vi "Base species cluster.vi"(11 "Base":string) -> (0 "ex":string, 1 "Base Color":u32, 2 "Base Array":bool[](array[boolean]), 3 "Base Species IDX":i32, 4 "Item":T1)   [LabVIEW 2018]
panel:
  out "R STD Level":dbl
  out "R Base Level":dbl
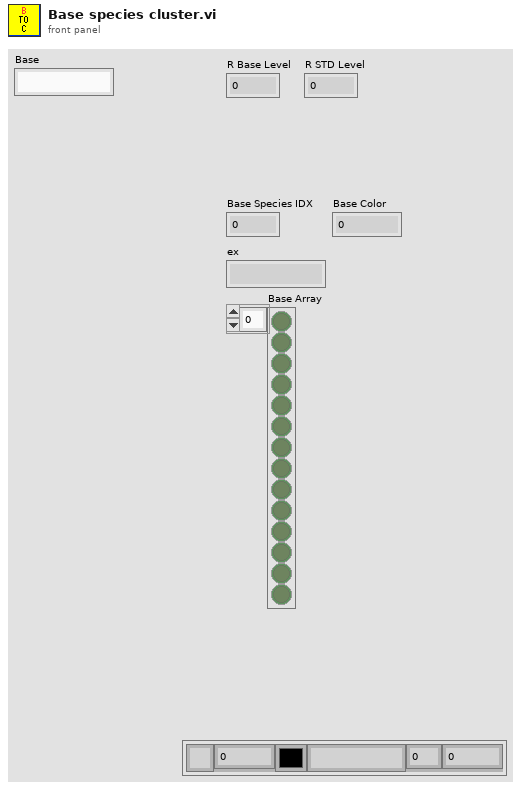
[diagram p1: front panel]
types:
  T1 = cluster{"Name":string, "Value":dbl, "Color":u32, "Name 2":string, "Value 2":dbl, "Value 3":dbl}
  T2 = cluster{"Base":string, dbl, u32, "y":string, i32, dbl}
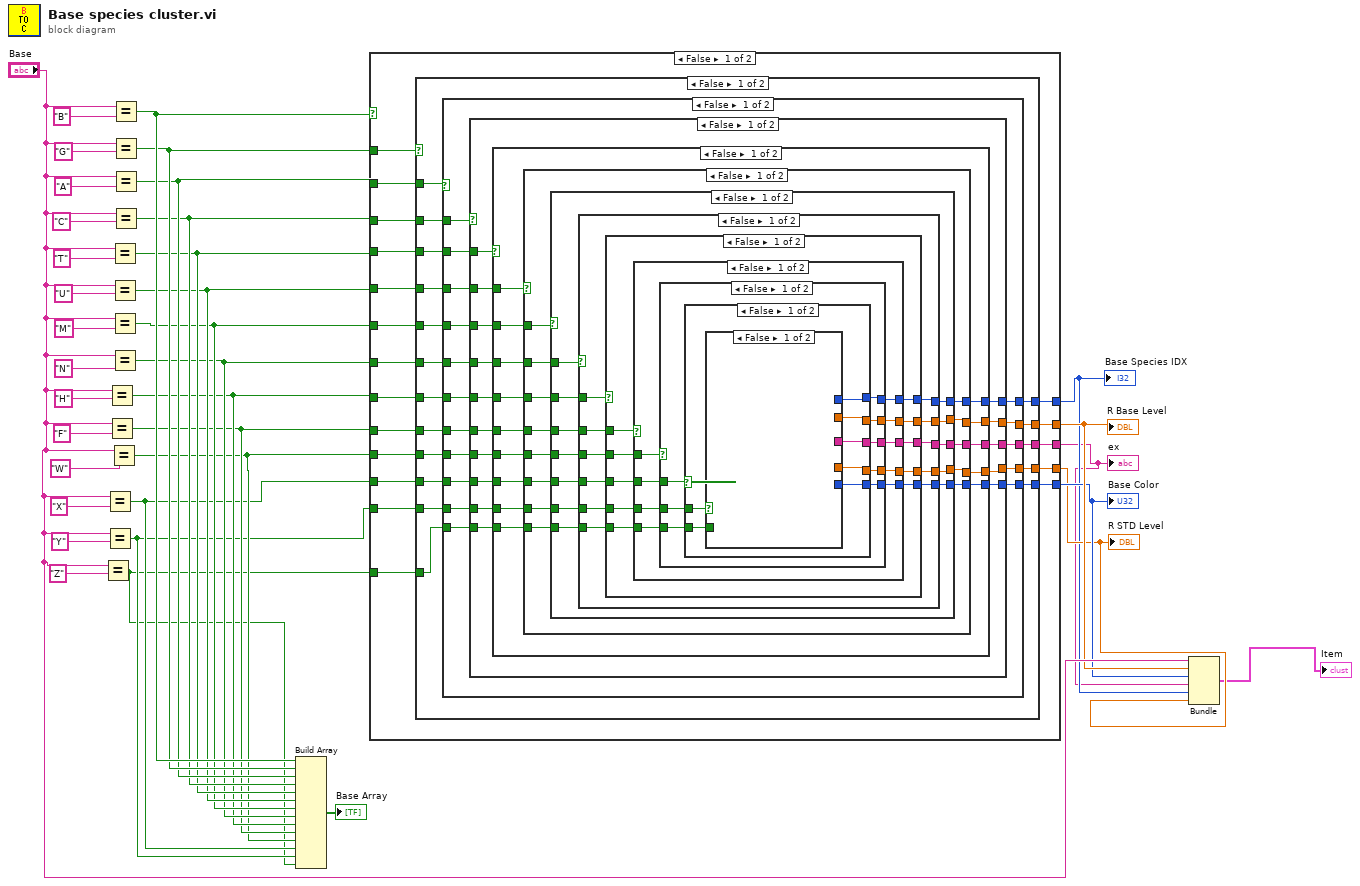
[diagram p0: block diagram]
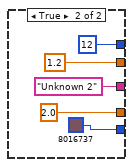
[diagram p2: hidden frame]
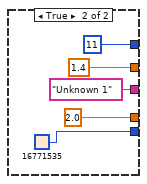
[diagram p3: hidden frame]
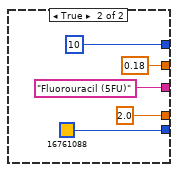
[diagram p4: hidden frame]
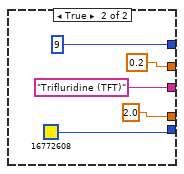
[diagram p5: hidden frame]
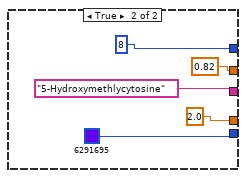
[diagram p6: hidden frame]
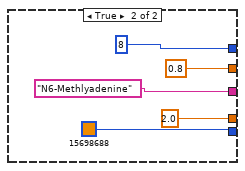
[diagram p7: hidden frame]
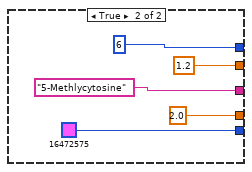
[diagram p8: hidden frame]
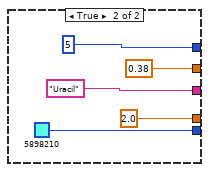
[diagram p9: hidden frame]
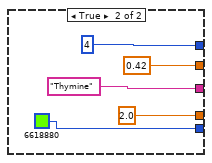
[diagram p10: hidden frame]
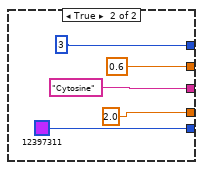
[diagram p11: hidden frame]
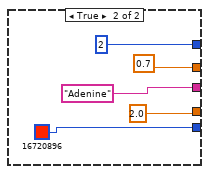
[diagram p12: hidden frame]
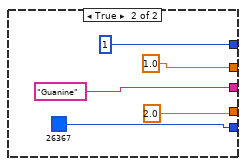
[diagram p13: hidden frame]
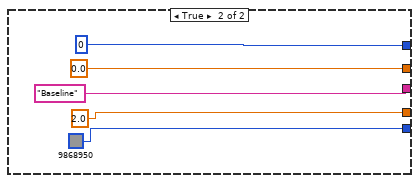
[diagram p14: hidden frame]
diagram:
  n1 = Equal?(x="Base", y="Z") -> (x = y?=w9:bool)
  n2 = Equal?(x="Base", y="X") -> (x = y?=w11:bool)
  n3 = Equal?(x="Base", y="Y") -> (x = y?=w10:bool)
  n4 = Equal?(x="Base", y="H") -> (x = y?=w14:bool)
  n5 = Equal?(x="Base", y="F") -> (x = y?=w13:bool)
  n6 = Equal?(x="Base", y="W") -> (x = y?=w12:bool)
  n7 = Equal?(x="Base", y="T") -> (x = y?=w18:bool)
  n8 = Equal?(x="Base", y="U") -> (x = y?=w17:bool)
  n9 = Equal?(x="Base", y="M") -> (x = y?=w16:bool)
  n10 = Equal?(x="Base", y="N") -> (x = y?=w15:bool)
  n11 = Equal?(x="Base", y="B") -> (x = y?=w22:bool)
  n12 = Equal?(x="Base", y="G") -> (x = y?=w21:bool)
  n13 = Equal?(x="Base", y="A") -> (x = y?=w20:bool)
  n14 = Equal?(x="Base", y="C") -> (x = y?=w19:bool)
  n15 = Build Array(w22, w21, w20, w19, w18, w17, w16, w15, w14, w13, w12, w11, w10, w9) -> (→"Base Array":bool[])
  n16 = case shown="False" w22 {
    tunnel: [w53 0] -> w3
    tunnel: w21 -> [w54 _]
    tunnel: [w52 "Baseline" ("y")] -> w2
    tunnel: w20 -> [w51 _]
    tunnel: w19 -> [w50 _]
    tunnel: w18 -> [w49 _]
    tunnel: w17 -> [w48 _]
    tunnel: w16 -> [w47 _]
    tunnel: w15 -> [w46 _]
    tunnel: w14 -> [w45 _]
    tunnel: w13 -> [w44 _]
    tunnel: w12 -> [w43 _]
    tunnel: w11 -> [w42 _]
    tunnel: w10 -> [w41 _]
    tunnel: w9 -> [w40 _]
    tunnel: [w39 u32 9868950] -> w5
    tunnel: [w38 0.0] -> w6
    tunnel: [w37 2.0] -> w4
    frame False {
      n17 = case shown="False" w54 {
        tunnel: [w71 1] -> w53
        tunnel: [w69 "Guanine" ("y")] -> w52
        tunnel: w51 -> [w70 _]
        tunnel: w50 -> [w68 _]
        tunnel: w49 -> [w67 _]
        tunnel: w48 -> [w66 _]
        tunnel: w47 -> [w65 _]
        tunnel: w46 -> [w64 _]
        tunnel: w45 -> [w63 _]
        tunnel: w44 -> [w62 _]
        tunnel: w43 -> [w61 _]
        tunnel: w42 -> [w60 _]
        tunnel: w41 -> [w59 _]
        tunnel: w40 -> [w58 _]
        tunnel: [w57 u32 26367] -> w39
        tunnel: [w56 1.0] -> w38
        tunnel: [w55 2.0] -> w37
        frame False {
          n18 = case shown="False" w70 {
            tunnel: [w86 2] -> w71
            tunnel: [w85 "Adenine" ("y")] -> w69
            tunnel: w68 -> [w87 _]
            tunnel: w67 -> [w84 _]
            tunnel: w66 -> [w83 _]
            tunnel: w65 -> [w82 _]
            tunnel: w64 -> [w81 _]
            tunnel: w63 -> [w80 _]
            tunnel: w62 -> [w79 _]
            tunnel: w61 -> [w78 _]
            tunnel: w60 -> [w77 _]
            tunnel: w59 -> [w76 _]
            tunnel: w58 -> [w75 _]
            tunnel: [w74 u32 16720896] -> w57
            tunnel: [w73 0.7] -> w56
            tunnel: [w72 2.0] -> w55
            frame False {
              n19 = case shown="False" w87 {
                tunnel: [w102 3] -> w86
                tunnel: [w100 "Cytosine"] -> w85
                tunnel: w84 -> [w101 _]
                tunnel: w83 -> [w99 _]
                tunnel: w82 -> [w98 _]
                tunnel: w81 -> [w97 _]
                tunnel: w80 -> [w96 _]
                tunnel: w79 -> [w95 _]
                tunnel: w78 -> [w94 _]
                tunnel: w77 -> [w93 _]
                tunnel: w76 -> [w92 _]
                tunnel: w75 -> [w91 _]
                tunnel: [w90 u32 12397311] -> w74
                tunnel: [w89 0.6] -> w73
                tunnel: [w88 2.0] -> w72
                frame False {
                  n20 = case shown="False" w101 {
                    tunnel: [w115 4] -> w102
                    tunnel: [w114 "Thymine"] -> w100
                    tunnel: w99 -> [w116 _]
                    tunnel: w98 -> [w113 _]
                    tunnel: w97 -> [w112 _]
                    tunnel: w96 -> [w111 _]
                    tunnel: w95 -> [w110 _]
                    tunnel: w94 -> [w109 _]
                    tunnel: w93 -> [w108 _]
                    tunnel: w92 -> [w107 _]
                    tunnel: w91 -> [w106 _]
                    tunnel: [w105 u32 6618880] -> w90
                    tunnel: [w104 0.42] -> w89
                    tunnel: [w103 2.0] -> w88
                    frame False {
                      n21 = case shown="False" w116 {
                        tunnel: [w128 5] -> w115
                        tunnel: [w127 "Uracil"] -> w114
                        tunnel: w113 -> [w129 _]
                        tunnel: w112 -> [w126 _]
                        tunnel: w111 -> [w125 _]
                        tunnel: w110 -> [w124 _]
                        tunnel: w109 -> [w123 _]
                        tunnel: w108 -> [w122 _]
                        tunnel: w107 -> [w121 _]
                        tunnel: w106 -> [w120 _]
                        tunnel: [w119 u32 5898210] -> w105
                        tunnel: [w118 0.38] -> w104
                        tunnel: [w117 2.0] -> w103
                        frame False {
                          n22 = case shown="False" w129 {
                            tunnel: [w140 6] -> w128
                            tunnel: [w139 "5-Methlycytosine"] -> w127
                            tunnel: w126 -> [w141 _]
                            tunnel: w125 -> [w138 _]
                            tunnel: w124 -> [w137 _]
                            tunnel: w123 -> [w136 _]
                            tunnel: w122 -> [w135 _]
                            tunnel: w121 -> [w134 _]
                            tunnel: w120 -> [w133 _]
                            tunnel: [w132 u32 16472575] -> w119
                            tunnel: [w131 1.2] -> w118
                            tunnel: [w130 2.0] -> w117
                            frame False {
                              n23 = case shown="False" w141 {
                                tunnel: [w151 8] -> w140
                                tunnel: [w150 "N6-Methlyadenine"] -> w139
                                tunnel: w138 -> [w152 _]
                                tunnel: w137 -> [w149 _]
                                tunnel: w136 -> [w148 _]
                                tunnel: w135 -> [w147 _]
                                tunnel: w134 -> [w146 _]
                                tunnel: w133 -> [w145 _]
                                tunnel: [w144 u32 15698688] -> w132
                                tunnel: [w143 0.8] -> w131
                                tunnel: [w142 2.0] -> w130
                                frame False {
                                n24 = case shown="False" w152 {
                                tunnel: [w162 8] -> w151
                                tunnel: [w161 "5-Hydroxymethlycytosine"] -> w150
                                tunnel: w149 -> [w160 _]
                                tunnel: w148 -> [w159 _]
                                tunnel: w147 -> [w158 _]
                                tunnel: w146 -> [w157 _]
                                tunnel: w145 -> [w156 _]
                                tunnel: [w155 u32 6291695] -> w144
                                tunnel: [w154 0.82] -> w143
                                tunnel: [w153 2.0] -> w142
                                frame False {
                                n25 = case shown="False" w160 {
                                tunnel: [w171 9] -> w162
                                tunnel: [w170 "Trifluridine (TFT)"] -> w161
                                tunnel: w159 -> [w169 _]
                                tunnel: w158 -> [w168 _]
                                tunnel: w157 -> [w167 _]
                                tunnel: w156 -> [w166 _]
                                tunnel: [w165 u32 16772608] -> w155
                                tunnel: [w163 0.2] -> w154
                                tunnel: [w164 2.0] -> w153
                                frame False {
                                n26 = case shown="False" w169 {
                                tunnel: [w178 10] -> w171
                                tunnel: [w177 "Fluorouracil (5FU)"] -> w170
                                tunnel: w168 -> [w179 _]
                                tunnel: w167 -> [w176 _]
                                tunnel: w166 -> [w175 _]
                                tunnel: [w174 u32 16761088] -> w165
                                tunnel: [w172 2.0] -> w164
                                tunnel: [w173 0.18] -> w163
                                frame False {
                                n27 = case shown="False" w179 {
                                tunnel: [w185 11] -> w178
                                tunnel: [w184 "Unknown 1"] -> w177
                                tunnel: w176 -> [w186 _]
                                tunnel: w175 -> [w183 _]
                                tunnel: [w182 u32 16771535] -> w174
                                tunnel: [w181 1.4] -> w173
                                tunnel: [w180 2.0] -> w172
                                frame False {
                                n28 = case shown="False" w186 {
                                tunnel: [w191 12] -> w185
                                tunnel: [w190 "Unknown 2"] -> w184
                                tunnel: w183 -> [w192 _]
                                tunnel: [w189 u32 8016737] -> w182
                                tunnel: [w188 1.2] -> w181
                                tunnel: [w187 2.0] -> w180
                                frame False {
                                n29 = case shown="False" w192 {
                                tunnel: [99 13] -> w191
                                tunnel: ["Z" "Unknown 3"] -> w190
                                tunnel: [u32 592137 u32 11776947] -> w189
                                tunnel: [1.6 1.6] -> w188
                                tunnel: [2.0 2.0] -> w187
                                frame False {
                                }
                                frame True {
                                }
                                }
                                }
                                frame True {
                                }
                                }
                                }
                                frame True {
                                }
                                }
                                }
                                frame True {
                                }
                                }
                                }
                                frame True {
                                }
                                }
                                }
                                frame True {
                                }
                                }
                                }
                                frame True {
                                }
                              }
                            }
                            frame True {
                            }
                          }
                        }
                        frame True {
                        }
                      }
                    }
                    frame True {
                    }
                  }
                }
                frame True {
                }
              }
            }
            frame True {
            }
          }
        }
        frame True {
        }
      }
    }
    frame True {
    }
  }
  "Base Species IDX" <- w3
  "ex" <- w2
  "Base Color" <- w5
  "R Base Level" <- w6
  "R STD Level" <- w4
  n30 = Bundle("Base"="Base", w6, w5, "y"=w2, w3, w4) -> (→"Item":T2)  [unwired: 1 in]
